vi "ComputeRowsCols.vi"(9 "error in (no error)":errorcluster, 10 "1-bit pixmap":T1) -> (0 "error out":errorcluster, 1 "#rows":i32, 2 "# cols":i32, 3 "origin":i32)   [LabVIEW 2026]
uses:
  Control 2.ctl
  Control 1.ctl
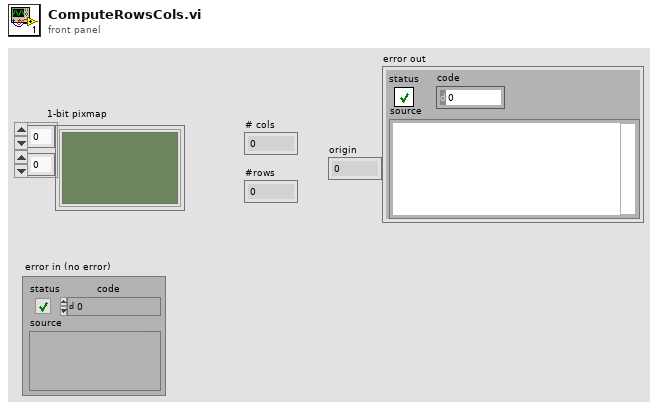
[diagram p1: front panel]
types:
  T1 = typedef "Control 2.ctl" = T2[][]
  T2 = typedef "Control 1.ctl" = bool
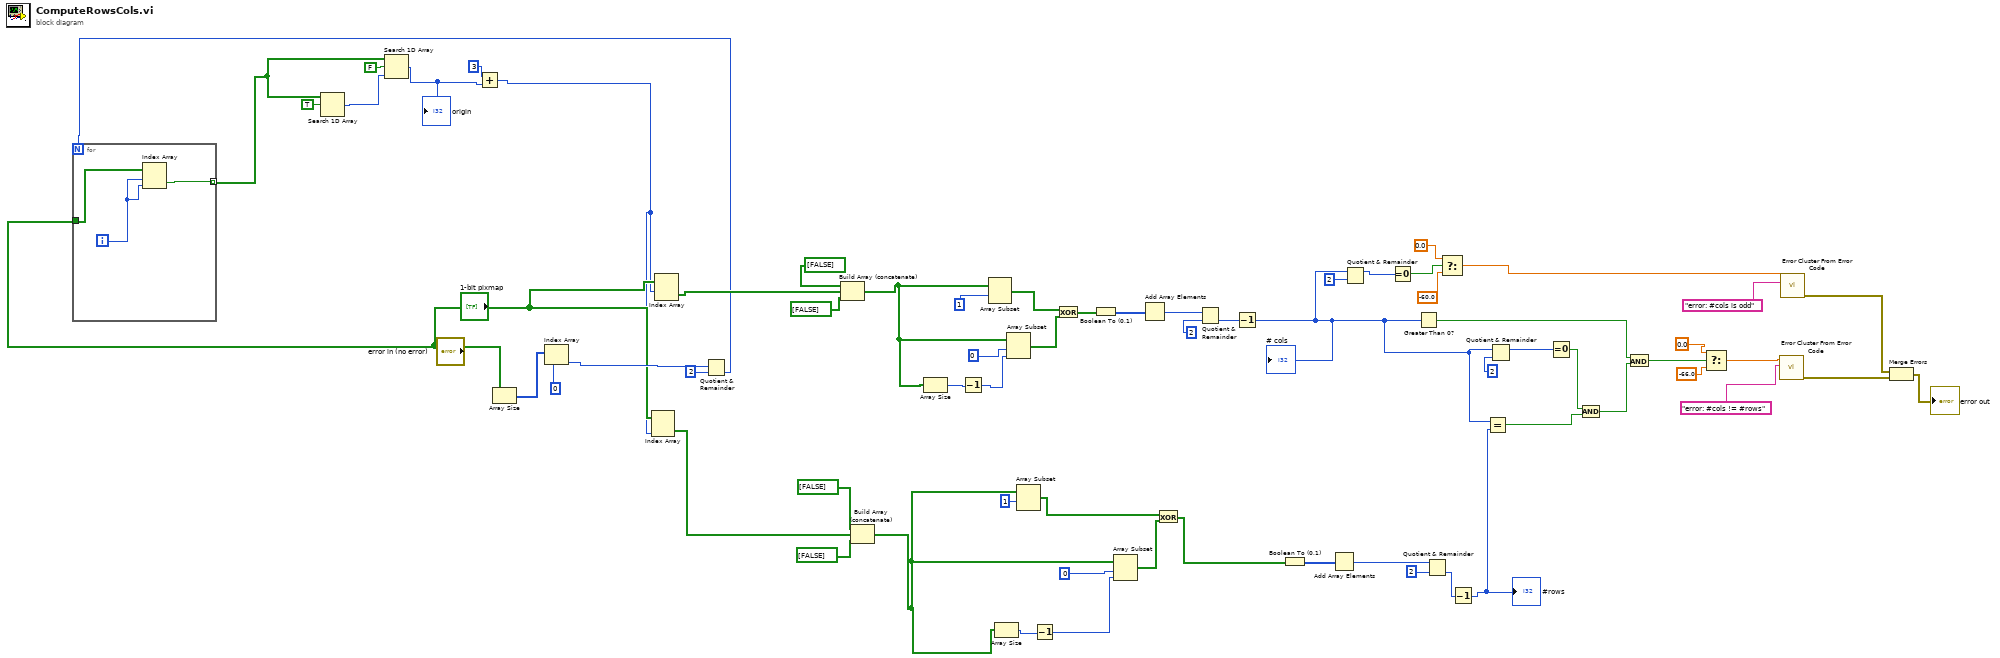
[diagram p0: block diagram]
diagram:
  n1 = Array Size(array="1-bit pixmap") -> (size(s)=w24:i32[])
  n2 = Index Array(array=w24, index=0) -> (element=w22:i32)
  n3 = Quotient & Remainder(x=w22, y=2) -> (floor(x/y)=w20:i32)  [unwired: 1 out]
  n4 = for {
    N: w20 -> [_]
    tunnel: "1-bit pixmap" -> [w69]
    tunnel: [w67] -> w18 mode=indexing
    i -> [w68]
    n5 = Index Array(array=w69, index (row)=w68, index (col)=w68) -> (element=w67:T2)
  }
  n6 = Search 1D Array(1D array=w18, element=T2 TRUE) -> (index of element=w16:i32)  [unwired: 1 in]
  n7 = Search 1D Array(1D array=w18, element=T2 FALSE, start index (0)=w16) -> (index of element=w15:i32)
  "origin" <- w15
  n8 = Add(x=3, y=w15) -> (x+y=w12:i32)
  n9 = Index Array(array="1-bit pixmap", index (col)=w12) -> (element=w41:T2[])  [unwired: 1 in]
  n10 = Index Array(array="1-bit pixmap", index (row)=w12) -> (element=w28:T2[])  [unwired: 1 in]
  n11 = Build Array (concatenate)(T2[] [FALSE] ("element"), w28, T2[] [FALSE] ("element")) -> (w25:T2[])
  n12 = Build Array (concatenate)(T2[] [FALSE] ("array"), w41, T2[] [FALSE] ("element")) -> (w52:T2[])
  n13 = Array Size(array=w25) -> (size(s)=w64:i32)
  n14 = Decrement(x=w64) -> (x-1=w26:i32)
  n15 = Array Subset(array=w25, index=1) -> (w61:T2[])  [unwired: 1 in]
  n16 = Array Size(array=w52) -> (size(s)=w53:i32)
  n17 = Array Subset(array=w25, index=0, length=w26) -> (w62:T2[])
  n18 = Array Subset(array=w52, index=1) -> (w49:T2[])  [unwired: 1 in]
  n19 = Decrement(x=w53) -> (x-1=w46:i32)
  n20 = Exclusive Or(1:w62, 2:w61) -> (0:w60:T2[])
  n21 = Boolean To (0,1)(Boolean=w60) -> (0, 1=w59:i16[])
  n22 = Array Subset(array=w52, index=0, length=w46) -> (w50:T2[])
  n23 = Add Array Elements(numeric array=w59) -> (sum=w58:i16)
  n24 = Exclusive Or(1:w50, 2:w49) -> (0:w48:T2[])
  n25 = Quotient & Remainder(x=w58, y=i16 2) -> (floor(x/y)=w56:i16)  [unwired: 1 out]
  n26 = Decrement(x=w56) -> (x-1=w10:i16)
  "# cols" <- w10
  n27 = Boolean To (0,1)(Boolean=w48) -> (0, 1=w47:i16[])
  n28 = Add Array Elements(numeric array=w47) -> (sum=w45:i16)
  n29 = Quotient & Remainder(x=w10, y=i16 2) -> (x-y*floor(x/y)=w5:i16)  [unwired: 1 out]
  n30 = Equal To 0?(x=w5) -> (x = 0?=w4:bool)
  n31 = Greater Than 0?(x=w10) -> (x > 0?=w35:bool)
  n32 = Quotient & Remainder(x=w45, y=i16 2) -> (floor(x/y)=w43:i16)  [unwired: 1 out]
  n33 = Select(t=0.0, s=w4, f=-60.0) -> (s? t:f=w6:dbl)
  n34 = Decrement(x=w43) -> (x-1=w40:i16)
  "#rows" <- w40
  n35 = Equal?(x=w10, y=w40) -> (x = y?=w37:bool)
  n36 = Quotient & Remainder(x=w10, y=i16 2) -> (x-y*floor(x/y)=w38:i16)  [unwired: 1 out]
  n37 = Equal To 0?(x=w38) -> (x = 0?=w36:bool)
  n38 = And(x=w36, y=w37) -> (x .and. y?=w34:bool)
  n39 = And(x=w35, y=w34) -> (x .and. y?=w33:bool)
  n40 = Select(t=0.0, s=w33, f=-66.0) -> (s? t:f=w30:dbl)
  n41 = call <vilib>:"Error Cluster From Error Code.vi"("error message (\"\")"="error: #cols != #rows" ("error message (\"\")"), "error code (0)"=w30) -> ("error out"=w3:errorcluster)  [unwired: 7 in]
  n42 = call <vilib>:"Error Cluster From Error Code.vi"("error message (\"\")"="error: #cols is odd" ("error message (\"\")"), "error code (0)"=w6) -> ("error out"=w2:errorcluster)  [unwired: 7 in]
  n43 = Merge Errors(w2, w3) -> (→"error out":errorcluster)
